vi "Write Builder Reference.vi"(8 "error in (no error)":errorcluster, 10 "new reference":T1, 11 "ToastBuilder in":refnum<class "ToastBuilder.lvclass">) -> (0 "error out":errorcluster, 3 "ToastBuilder out":refnum<class "ToastBuilder.lvclass">)   [LabVIEW 2026, in "ToastNotification.lvlib" / "ToastBuilder.lvclass"]
doc: "Private native data-member write accessor for Builder Reference. Store the supplied handle and pass the class and error through. Does not release a replaced handle or clone the new one. The method acquiring or replacing a handle is responsible for its lifetime. Use through the class property node."
uses:
  ToastBuilder.lvclass
  Builder Reference.ctl
  C:/Users/loicw/Documents/LabVIEW/ToastNotifications/Sources/bins/Microsoft.Toolkit.Uwp.Notifications.dll
  bins/Microsoft.Toolkit.Uwp.Notifications.dll
  ToastBuilder.lvclass/ToastBuilder.ctl
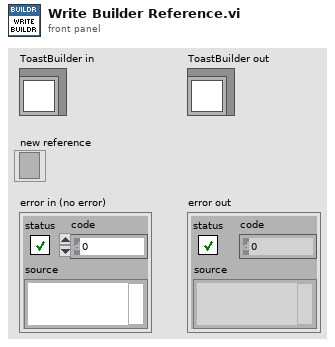
[diagram p1: front panel]
types:
  T1 = typedef "ToastNotification.lvlib/ToastBuilder.lvclass/Builder Reference.ctl" = refnum<k24>
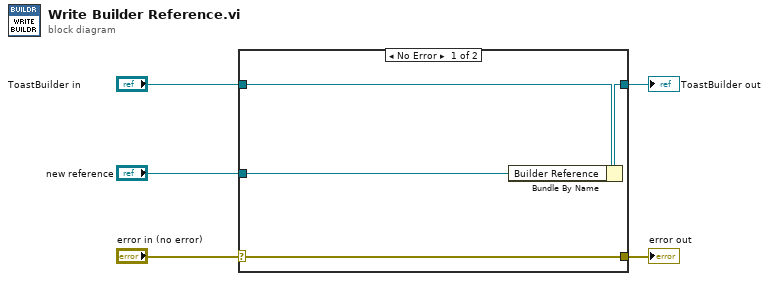
[diagram p0: block diagram]
diagram:
  n1 = case shown="No Error" "error in (no error)" {
    selector: "error in (no error)" -> [w9 w10]
    tunnel: [w9 w10] -> w4
    tunnel: [w7 w11] -> w2
    tunnel: "ToastBuilder in" -> [w8 w11]
    tunnel: "new reference" -> [w6 _]
    frame No Error {
      n2 = Bundle By Name(cluster=w8, "Builder Reference"=w6) -> (w7:refnum<class "ToastBuilder.lvclass">)
    }
    frame Error {
    }
  }
  "error out" <- w4
  "ToastBuilder out" <- w2
